vi "conf FCC Main EIRP Measurement.vi"(8 "error in (no error)":errorcluster, 11 "SA Measurement in":refnum<class "SA Measurement.lvclass">) -> (0 "error out":errorcluster, 3 "SA Measurement out":refnum<class "SA Measurement.lvclass">)   [LabVIEW 2023, in "Spectrum Analyzer.lvlib" / "SA Measurement.lvclass"]
uses:
  SA Measurement.lvclass
  TYPE DEFINITION/TYPE Measurement Window Mode.ctl
  TYPE DEFINITION/TYPE RBW and VBW Select.ctl
  TYPE DEFINITION/TYPE Average Mode Select.ctl
  SA Measurement.lvclass/SA Measurement.ctl
  Interface_Spectrum/Interface_Spectrum.lvclass
  Spectrum Analyzer.lvlib
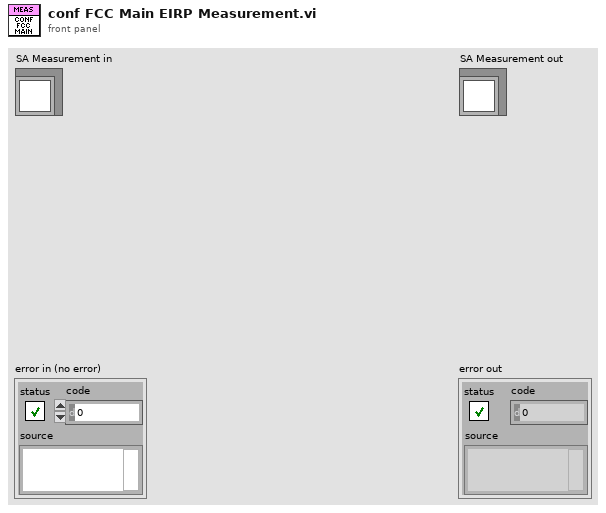
[diagram p1: front panel]
types:
  T1 = typedef "Spectrum Analyzer.lvlib/TYPE Average Mode Select.ctl" = enum16{"Linear(Voltage Avg)", "Video(Log)", "Power"}
  T2 = enum16{"TX Channel", "Adjacent Channel", "Alternate Channel"}
  T3 = typedef "Spectrum Analyzer.lvlib/TYPE RBW and VBW Select.ctl" = enum16{"Res BW", "Video BW"}
  T4 = typedef "Spectrum Analyzer.lvlib/TYPE Measurement Window Mode.ctl" = enum16{"ACPower", "CPOWer", "MCACpower", "OBANdwidth", "OBWidth", "CN", "CN0"}
  T5 = typedef "Spectrum Analyzer.lvlib/TYPE Y-axis Unit.ctl" = enum16{"dBm", "dBmV", "dBuV", "dBpW", "Volt", "Ampere", "Watt"}
  T6 = typedef "Spectrum Analyzer.lvlib/TYPE Reference Level and Atten Param.ctl" = cluster{"Reference Level":dbl, "Atten":i32, "Atten Auto?":bool, "Reference Level Offset":dbl}
  T7 = typedef "Spectrum Analyzer.lvlib/TYPE Display Trace Mode Select.ctl" = enum16{"Clear Write", "Max Hold", "Min Hold", "Average", "View"}
  T8 = typedef "Spectrum Analyzer.lvlib/TYPE Detect Mode Select.ctl" = enum16{"Det Auto (Normal)", "Auto Peak", "Positive Peak", "Negative Peak", "Sample", "RMS", "Average", "Quasipeak", "CISPR Average", "RMS Average"}
  T9 = cluster{"Trace Mode":T7, "Detector Type":T8, "Detect Auto?":bool}[]
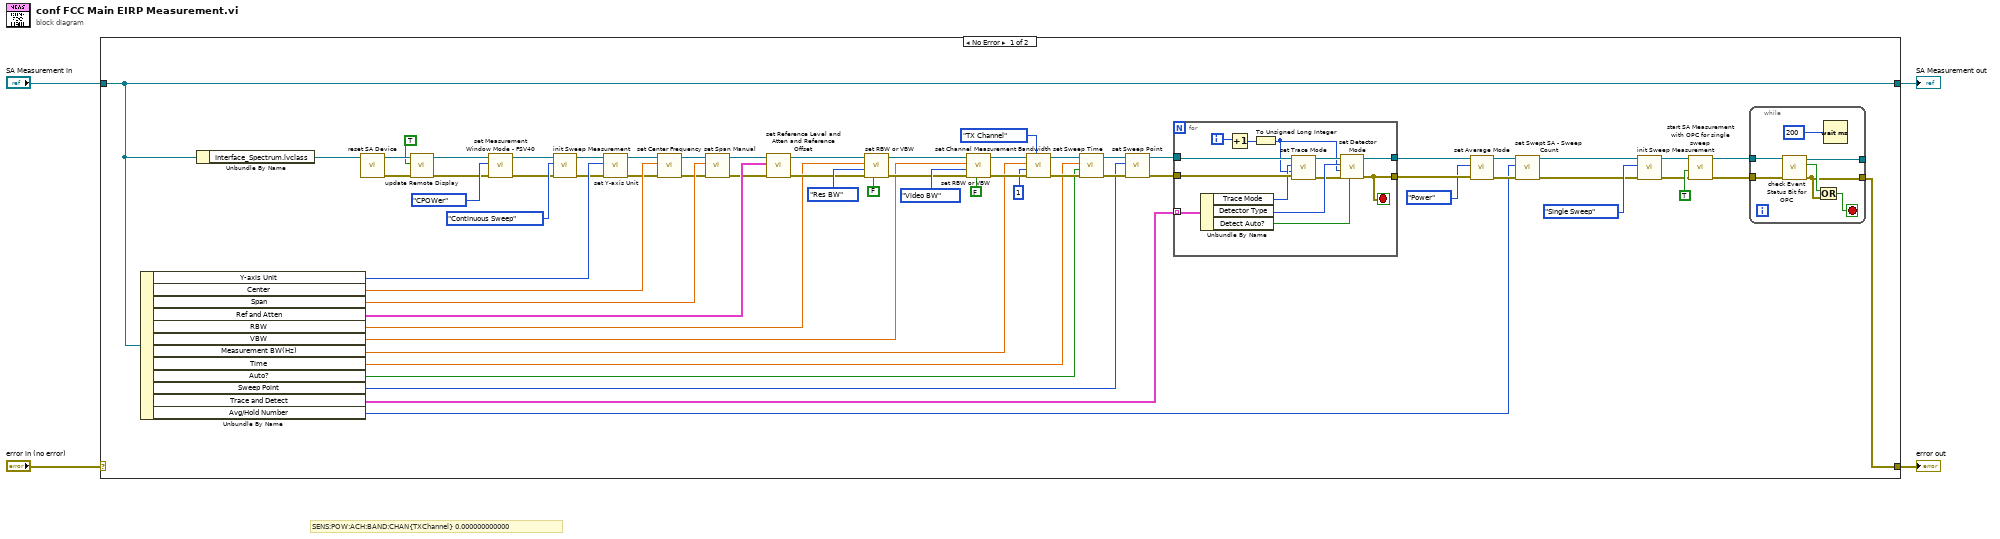
[diagram p0: block diagram]
diagram:
  # "SENS:POW:ACH:BAND:CHAN{TXChannel} 0.000000000000"
  n1 = case shown="No Error" "error in (no error)" {
    selector: "error in (no error)" -> [_ w89]
    tunnel: [w20 w89] -> w3
    tunnel: [w65 w88] -> w1
    tunnel: "SA Measurement in" -> [w65 w88]
    frame No Error {
      n2 = Unbundle By Name(w65) -> ("Y-axis Unit"=w64:T5, "Center"=w61:dbl, "Span"=w60:dbl, "Ref and Atten"=w51:T6, "RBW"=w46:dbl, "VBW"=w45:dbl, "Measurement BW(Hz)"=w42:dbl, "Time"=w37:dbl, "Auto?"=w36:bool, "Sweep Point"=w33:u32, "Trace and Detect"=w30:T9, "Avg/Hold Number"=w24:u32)
      n3 = Unbundle By Name(w65) -> ("Interface_Spectrum.lvclass"=w67:refnum<class "Interface_Spectrum.lvclass">)
      n4 = call-dynamic "reset SA Device.vi"("Interface_Spectrum in"=w67) -> ("error out"=w18:errorcluster, "Interface_Spectrum out"=w19:refnum<class "Interface_Spectrum.lvclass">)  [unwired: 9 in]
      n5 = call-dynamic "update Remote Display.vi"("error in (no error)"=w18, "Remote Display On?"=TRUE, "Interface_Spectrum in"=w19) -> ("error out"=w16:errorcluster, "Interface_Spectrum out"=w17:refnum<class "Interface_Spectrum.lvclass">)  [unwired: 7 in]
      n6 = call-dynamic "set Measurement Window Mode - FSV40.vi"("error in (no error)"=w16, "Measurement Window Mode"=TYPE_Measurement_Window_Mode."CPOWer", "Interface_Spectrum in"=w17) -> ("error out"=w12:errorcluster, "Interface_Spectrum out"=w13:refnum<class "Interface_Spectrum.lvclass">)  [unwired: 7 in]
      n7 = call-dynamic "init Sweep Measurement.vi"("error in (no error)"=w12, "Sweep Measurement Mode"=enum16{"Single Sweep", "Continuous Sweep"}."Continuous Sweep", "Interface_Spectrum in"=w13) -> ("error out"=w10:errorcluster, "Interface_Spectrum out"=w11:refnum<class "Interface_Spectrum.lvclass">)  [unwired: 7 in]
      n8 = call-dynamic "set Y-axis Unit.vi"("error in (no error)"=w10, "Y-axis Unit"=w64, "Interface_Spectrum in"=w11) -> ("error out"=w59:errorcluster, "Interface_Spectrum out"=w63:refnum<class "Interface_Spectrum.lvclass">)  [unwired: 7 in]
      n9 = call-dynamic "set Center Frequency.vi"("error in (no error)"=w59, "Center Frequency (Hz)"=w61, "Interface_Spectrum in"=w63) -> ("error out"=w58:errorcluster, "Interface_Spectrum out"=w62:refnum<class "Interface_Spectrum.lvclass">)  [unwired: 7 in]
      n10 = call-dynamic "set Span Manual.vi"("error in (no error)"=w58, "Span (Hz)"=w60, "Interface_Spectrum in"=w62) -> ("error out"=w49:errorcluster, "Interface_Spectrum out"=w50:refnum<class "Interface_Spectrum.lvclass">)  [unwired: 7 in]
      n11 = call-dynamic "set Reference Level and Atten and Reference Offset.vi"("error in (no error)"=w49, "Reference Level, Atten, Reference Offset"=w51, "Interface_Spectrum in"=w50) -> ("error out"=w47:errorcluster, "Interface_Spectrum out"=w48:refnum<class "Interface_Spectrum.lvclass">)  [unwired: 7 in]
      n12 = call-dynamic "set RBW or VBW.vi"("BW Auto?"=FALSE, "error in (no error)"=w47, "BW Type"=TYPE_RBW_and_VBW_Select."Res BW", "BW Value (Hz)"=w46, "Interface_Spectrum in"=w48) -> ("error out"=w52:errorcluster, "Interface_Spectrum out"=w53:refnum<class "Interface_Spectrum.lvclass">)  [unwired: 5 in]
      n13 = call-dynamic "set RBW or VBW.vi"("BW Auto?"=FALSE, "error in (no error)"=w52, "BW Type"=TYPE_RBW_and_VBW_Select."Video BW", "BW Value (Hz)"=w45, "Interface_Spectrum in"=w53) -> ("error out"=w43:errorcluster, "Interface_Spectrum out"=w44:refnum<class "Interface_Spectrum.lvclass">)  [unwired: 5 in]
      n14 = call-dynamic "set Channel Measurement Bandwidth.vi"("Target Channel Type"=T2."TX Channel", "error in (no error)"=w43, "TX Channel Index"=1, "Channel BandWidth (Hz)"=w42, "Interface_Spectrum in"=w44) -> ("error out"=w38:errorcluster, "Interface_Spectrum out"=w39:refnum<class "Interface_Spectrum.lvclass">)  [unwired: 5 in]
      n15 = call-dynamic "set Sweep Time.vi"("error in (no error)"=w38, "Sweep Time Auto?"=w36, "Sweep Time(sec)"=w37, "Interface_Spectrum in"=w39) -> ("error out"=w34:errorcluster, "Interface_Spectrum out"=w35:refnum<class "Interface_Spectrum.lvclass">)  [unwired: 6 in]
      n16 = call-dynamic "set Sweep Point.vi"("error in (no error)"=w34, "Sweep Point"=w33, "Interface_Spectrum in"=w35) -> ("error out"=w31:errorcluster, "Interface_Spectrum out"=w32:refnum<class "Interface_Spectrum.lvclass">)  [unwired: 7 in]
      n17 = for {
        tunnel: w32 -> [w86]
        tunnel: w31 -> [w85]
        tunnel: w30 -> [w87] mode=indexing
        tunnel: [w75] -> w26
        tunnel: [w76] -> w27
        i -> [w84]
        stop <- w75 stop-if-true
        n18 = Unbundle By Name(w87) -> ("Trace Mode"=w82:T7, "Detector Type"=w80:T8, "Detect Auto?"=w77:bool)
        n19 = Increment(x=w84) -> (x+1=w83:i32)
        n20 = To Unsigned Long Integer(number=w83) -> (unsigned 32bit integer=w78:u32)
        n21 = call-dynamic "set Trace Mode.vi"("error in (no error)"=w85, "Trace Index"=w78, "Trace Mode"=w82, "Interface_Spectrum in"=w86) -> ("error out"=w79:errorcluster, "Interface_Spectrum out"=w81:refnum<class "Interface_Spectrum.lvclass">)  [unwired: 6 in]
        n22 = call-dynamic "set Detector Mode.vi"("Detect Auto?"=w77, "error in (no error)"=w79, "Trace Index"=w78, "Detector Type"=w80, "Interface_Spectrum in"=w81) -> ("error out"=w75:errorcluster, "Interface_Spectrum out"=w76:refnum<class "Interface_Spectrum.lvclass">)  [unwired: 5 in]
      }
      n23 = call-dynamic "set Average Mode.vi"("error in (no error)"=w26, "Average Mode"=TYPE_Average_Mode_Select."Power", "Interface_Spectrum in"=w27) -> ("error out"=w28:errorcluster, "Interface_Spectrum out"=w29:refnum<class "Interface_Spectrum.lvclass">)  [unwired: 7 in]
      n24 = call-dynamic "set Swept SA - Sweep Count.vi"("error in (no error)"=w28, "Sweep Count"=w24, "Interface_Spectrum in"=w29) -> ("error out"=w7:errorcluster, "Interface_Spectrum out"=w8:refnum<class "Interface_Spectrum.lvclass">)  [unwired: 7 in]
      n25 = call-dynamic "init Sweep Measurement.vi"("error in (no error)"=w7, "Sweep Measurement Mode"=enum16{"Single Sweep", "Continuous Sweep"}."Single Sweep", "Interface_Spectrum in"=w8) -> ("error out"=w5:errorcluster, "Interface_Spectrum out"=w6:refnum<class "Interface_Spectrum.lvclass">)  [unwired: 7 in]
      n26 = call-dynamic "start SA Measurement with OPC for single sweep.vi"("error in (no error)"=w5, "with OPC?"=TRUE, "Interface_Spectrum in"=w6) -> ("error out"=w21:errorcluster, "Interface_Spectrum out"=w22:refnum<class "Interface_Spectrum.lvclass">)  [unwired: 7 in]
      n27 = while {
        tunnel: w22 -> [w74]
        tunnel: w21 -> [w73]
        tunnel: [w70] -> w20
        tunnel: [w69] -> _
        stop <- w71 stop-if-true
        n28 = call-dynamic "check Event Status Bit for OPC.vi"("error in (no error)"=w73, "Interface_Spectrum in"=w74) -> ("error out"=w70:errorcluster, "OPC Bit Changed?"=w72:bool, "Interface_Spectrum out"=w69:refnum<class "Interface_Spectrum.lvclass">)  [unwired: 7 in]
        n29 = Or(x=w72, y=w70) -> (x .or. y?=w71:bool)
        n30 = Wait (ms)(milliseconds to wait=u32 200) -> ()  [unwired: 1 out]
      }
    }
    frame Error {
    }
  }
  "error out" <- w3
  "SA Measurement out" <- w1
